vi "test tools list mcp names.vi"(8 "error in (no error)":errorcluster) -> (0 "error out":errorcluster, 3 "body":string)   [LabVIEW 2020, in "MCP Server tests.lvlib"]
doc: "tools/list names the inputs of a tool by their MCP names: a control label with upper case letters, spaces, brackets or special characters is lower cased and every character that is not a-z, 0-9, _ or - becomes _. fake_tool_special_labels has the required inputs Length (mm) and Factor #1 & 50%, which must be listed as length__mm_ and factor__1___50_ in properties and in required, and every name there must match ^[a-zA-Z0-9_-]{1,64}$."
uses:
  MCP Server tests.lvlib
  bd26dd9c-eeff-42d0-bbf2-bbcb6f80b1ee.vi
  <vilib>/JDP Science/JSONtext/Next JSON Value.vi
  <vilib>/JDP Science/JSONtext/String Subset.vi
  <vilib>/JDP Science/JSONtext/Parsing/Advance past next JSON Value (inlined COPY).vi
  <vilib>/JDP Science/JSONtext/Parsing/Advance past whitespace.vi
  <vilib>/JDP Science/JSONtext/Parsing/Advance past String.vi
  <vilib>/JDP Science/JSONtext/Parsing/Advance past Number.vi
  <vilib>/JDP Science/JSONtext/Parsing/Advance past Line Ending.vi
  <vilib>/JDP Science/JSONtext/Parsing/Parse Full Path or Item Name.vi
  <vilib>/JDP Science/JSONtext/Parsing/Advance past Array.vi
  <vilib>/JDP Science/JSONtext/Parsing/Advance past Object.vi
  <vilib>/JDP Science/JSONtext/support/Error Cluster From Code.vi
  <vilib>/JDP Science/JSONtext/Offset/Find Item Locations by Path.vi
  <vilib>/JDP Science/JSONtext/JSON text to Variant.vi
  <vilib>/JDP Science/JSONtext/LVClass Serializer/JSONtext LVClass Serializer.lvclass
  <vilib>/addons/_JKI Toolkits/Caraya/classes/Test/Test.lvclass
  <vilib>/JDP Science/JSONtext/JSONtext.lvlib
  <vilib>/addons/_JKI Toolkits/Caraya/classes/Assert/Assert.lvclass
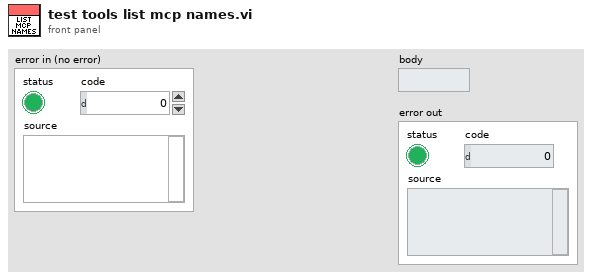
[diagram p1: front panel]
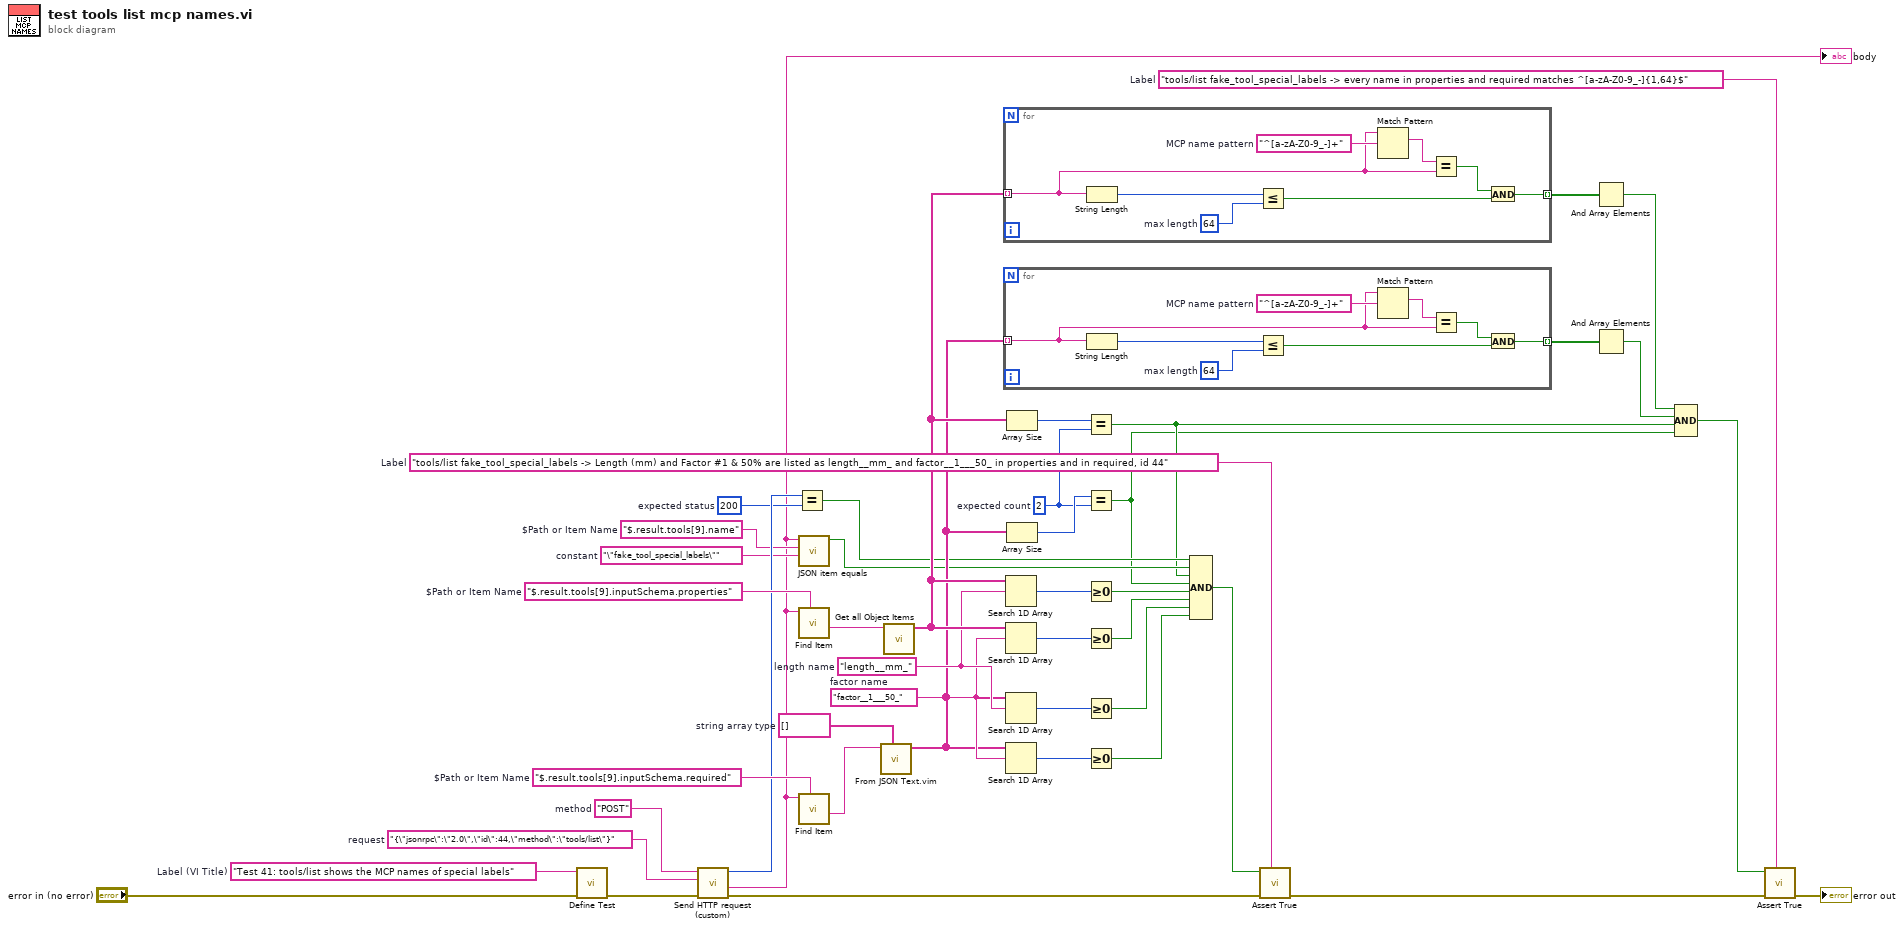
[diagram p0: block diagram]
diagram:
  w3 = "tools/list fake_tool_special_labels -> every name in properties and required matches ^[a-zA-Z0-9_-]{1,64}$"  # Label
  w6 = "tools/list fake_tool_special_labels -> Length (mm) and Factor #1 & 50% are listed as length__mm_ and factor__1___50_ in properties and in required, id 44"  # Label
  w29 = "factor__1___50_"  # factor name
  w30 = "length__mm_"  # length name
  w22 = 2  # expected count
  w32 = string[] []  # string array type
  w39 = "$.result.tools[9].inputSchema.required"  # $Path or Item Name
  w40 = "$.result.tools[9].inputSchema.properties"  # $Path or Item Name
  w35 = "\"fake_tool_special_labels\""  # constant
  w36 = "$.result.tools[9].name"  # $Path or Item Name
  w37 = 200  # expected status
  w42 = "{\"jsonrpc\":\"2.0\",\"id\":44,\"method\":\"tools/list\"}"  # request
  w43 = "POST"  # method
  w45 = "Test 41: tools/list shows the MCP names of special labels"  # Label (VI Title)
  n1 = call <vilib>:"Define Test.vi"("error in (no error)"="error in (no error)", "Label (VI Title)"=w45) -> ("error out"=w41:errorcluster)  [unwired: 8 in, 1 out]
  n2 = call "Send HTTP request (custom).vi"("error in (no error)"=w41, "request"=w42, "method"=w43) -> ("error out"=w7:errorcluster, "response"=w2:string, "status code"=w38:i32)  [unwired: 5 in, 1 out]
  "body" <- w2
  n3 = Equal?(x=w38, y=w37) -> (x = y?=w18:bool)
  n4 = call "JSON item equals.vi"("expected"=w35, "path"=w36, "JSON"=w2) -> ("equal?"=w17:bool)  [unwired: 6 in, 2 out]
  n5 = call <vilib>:"Find Item.vi"("$Path or Item Name"=w40, "JSON"=w2) -> ("<JSON>"=w34:string)  [unwired: 6 in, 3 out]
  n6 = call <vilib>:"Find Item.vi"("$Path or Item Name"=w39, "JSON"=w2) -> ("<JSON>"=w33:string)  [unwired: 6 in, 3 out]
  n7 = call "From JSON Text.vim"("Data Type and Default Value"=w32, "JSON"=w33) -> ("Data out"=w28:string[])  [unwired: 8 in, 1 out]
  n8 = call <vilib>:"Get all Object Items.vi"("JSON"=w34) -> ("Item Names"=w31:string[])  [unwired: 7 in, 3 out]
  n9 = for {
    tunnel: w31 -> [w49] mode=indexing
    tunnel: [w46] -> w24 mode=indexing
    w51 = 64  # max length
    w53 = "^[a-zA-Z0-9_-]+"  # MCP name pattern
    n10 = String Length(string=w49) -> (length=w52:i32)
    n11 = Less Or Equal?(x=w52, y=w51) -> (x <= y?=w47:bool)
    n12 = Match Pattern(string=w49, regular expression=w53) -> (match substring=w50:string)  [unwired: 1 in, 3 out]
    n13 = Equal?(x=w50, y=w49) -> (x = y?=w48:bool)
    n14 = And(x=w48, y=w47) -> (x .and. y?=w46:bool)
  }
  n15 = for {
    tunnel: w28 -> [w57] mode=indexing
    tunnel: [w54] -> w19 mode=indexing
    w59 = 64  # max length
    w61 = "^[a-zA-Z0-9_-]+"  # MCP name pattern
    n16 = String Length(string=w57) -> (length=w60:i32)
    n17 = Less Or Equal?(x=w60, y=w59) -> (x <= y?=w55:bool)
    n18 = Match Pattern(string=w57, regular expression=w61) -> (match substring=w58:string)  [unwired: 1 in, 3 out]
    n19 = Equal?(x=w58, y=w57) -> (x = y?=w56:bool)
    n20 = And(x=w56, y=w55) -> (x .and. y?=w54:bool)
  }
  n21 = Search 1D Array(1D array=w31, element=w30) -> (index of element=w26:i32)  [unwired: 1 in]
  n22 = Search 1D Array(1D array=w31, element=w29) -> (index of element=w25:i32)  [unwired: 1 in]
  n23 = Search 1D Array(1D array=w28, element=w30) -> (index of element=w21:i32)  [unwired: 1 in]
  n24 = Search 1D Array(1D array=w28, element=w29) -> (index of element=w20:i32)  [unwired: 1 in]
  n25 = Array Size(array=w31) -> (size(s)=w27:i32)
  n26 = Array Size(array=w28) -> (size(s)=w23:i32)
  n27 = Equal?(x=w27, y=w22) -> (x = y?=w10:bool)
  n28 = Equal?(x=w23, y=w22) -> (x = y?=w9:bool)
  n29 = Greater Or Equal To 0?(x=w26) -> (x >= 0?=w16:bool)
  n30 = Greater Or Equal To 0?(x=w25) -> (x >= 0?=w15:bool)
  n31 = Greater Or Equal To 0?(x=w21) -> (x >= 0?=w14:bool)
  n32 = Greater Or Equal To 0?(x=w20) -> (x >= 0?=w13:bool)
  n33 = Compound Arithmetic op=AND(w18, w17, w10, w9, w16, w15, w14, w13) -> (w8:bool)
  n34 = call <vilib>:"Assert True.vi"("Label"=w6, "error in (no error)"=w7, "True?"=w8) -> ("error out"=w4:errorcluster)  [unwired: 7 in, 1 out]
  n35 = And Array Elements(Boolean array=w24) -> (logical AND=w12:bool)
  n36 = And Array Elements(Boolean array=w19) -> (logical AND=w11:bool)
  n37 = Compound Arithmetic op=AND(w12, w11, w10, w9) -> (w5:bool)
  n38 = call <vilib>:"Assert True.vi"("Label"=w3, "error in (no error)"=w4, "True?"=w5) -> ("error out"=→"error out":errorcluster)  [unwired: 7 in, 1 out]
